vi "New MS IDX VI.vi"(8 "Sample Sequence":string, 9 "Direction":string="5f¨3'", 11 "Base Number":i32[](array[numeric])) -> (3 "Array":i32[](array[numeric]))   [LabVIEW 2018]
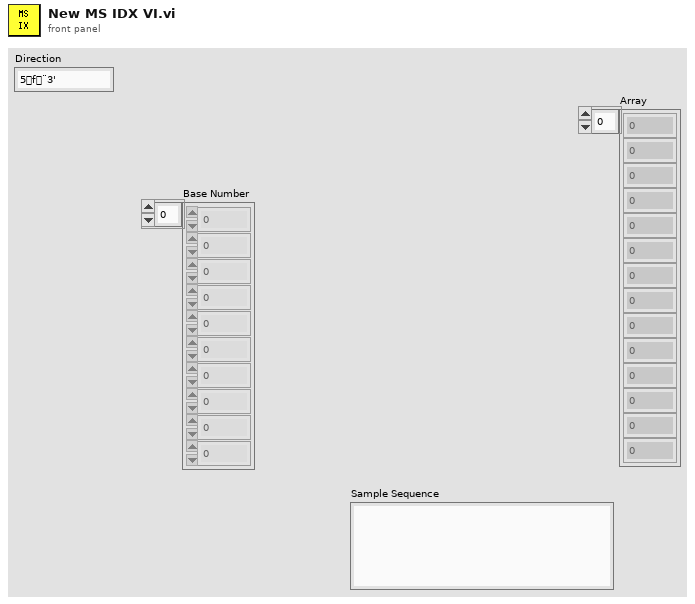
[diagram p1: front panel]
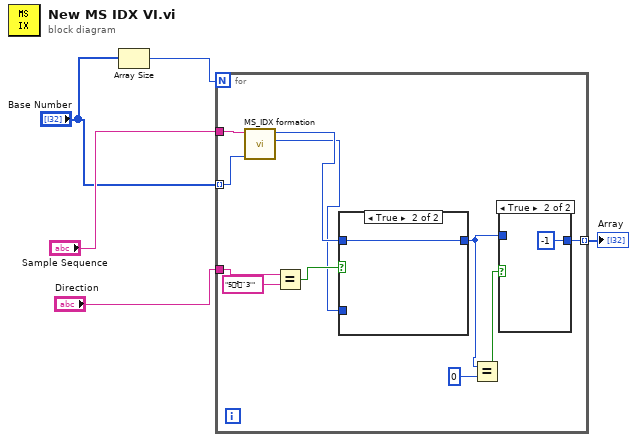
[diagram p0: block diagram]
diagram:
  n1 = Array Size(array="Base Number") -> (size(s)=w5:i32)
  n2 = for {
    N: w5 -> [_]
    tunnel: "Sample Sequence" -> [w16]
    tunnel: "Base Number" -> [w15] mode=indexing
    tunnel: "Direction" -> [w14]
    tunnel: [w9] -> w2 mode=indexing
    n3 = call "MS_IDX formation.vi"("AS_ISX"=w15, "Sample sequnce"=w16) -> ("MS_IXD3"=w10:i32, "MS_IXD5"=w11:i32)  [unwired: 7 in, 1 out]
    n4 = Equal?(x=w14, y="5f¨3'") -> (x = y?=w12:bool)
    n5 = case shown="True" w12 {
      tunnel: w11 -> [_ w20]
      tunnel: w10 -> [w19 _]
      tunnel: [w19 w20] -> w8
      frame False {
      }
      frame True {
      }
    }
    n6 = Equal?(x=w8, y=0) -> (x = y?=w6:bool)
    n7 = case shown="True" w6 {
      tunnel: w8 -> [w17 _]
      tunnel: [w17 -1 ("MS_IXD5")] -> w9
      frame False {
      }
      frame True {
      }
    }
  }
  "Array" <- w2
